vi "ELLjog.vi"() -> ()   [LabVIEW 2019]
uses:
  C:/Users/gboedecker/Downloads/ELL_Example/ELL/Thorlabs.Elliptec.ELLO_DLL.dll
  ELL_Example/ELL/Thorlabs.Elliptec.ELLO_DLL.dll
panel:
  out "Position":dbl format="%#.3f"
  in  "Enum":enum16{"None", "Button1", "Button2"}(ring)
  in  "Clockwise":bool
  in  "?":bool
  in  "Counter Clockwise":bool
  out "Connected":bool
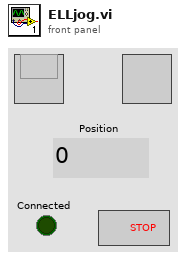
[diagram p1: front panel]
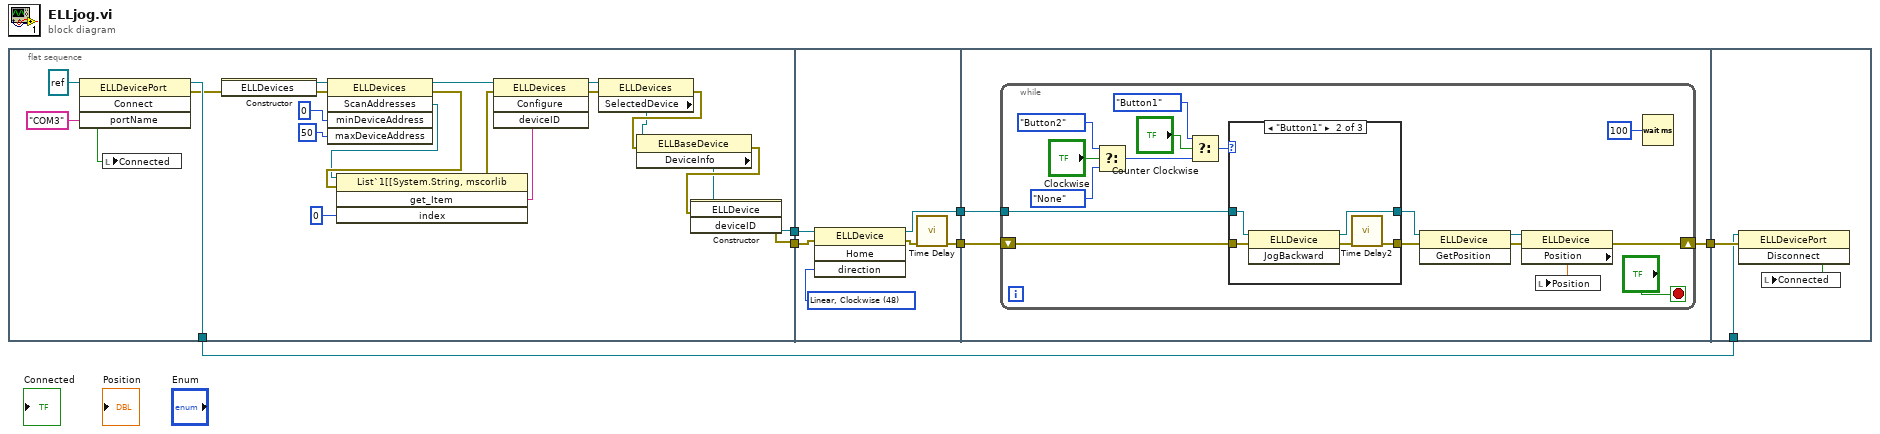
[diagram p0: block diagram]
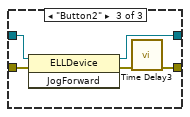
[diagram p3: hidden frame]
diagram:
  n1 = flat-sequence {
    tunnel: [w29] -> w3
    tunnel: [w28] -> w2
    tunnel: [w8] -> w1
    tunnel: [w35] -> w5
    tunnel: [w30] -> w4
    tunnel: w3 -> [w33]
    tunnel: w2 -> [w32]
    tunnel: [w38] -> w6
    tunnel: w5 -> [w37]
    tunnel: w4 -> [w36]
    tunnel: w6 -> [w69]
    tunnel: w1 -> [w68]
    frame #0 {
      n2 = invoke class="ELLDevicePort" method="Connect"(reference=refnum<k24> refnum, "portName"="COM3") -> (reference out=w8:refnum<k24>, error out=w7:errorcluster, "Connect"=w11:bool)  [unwired: 2 in, 1 out]
      n3 = local write "Connected"(w11) -> ()
      n4 = constructor class="ELLDevices"(error in=w7) -> (reference out=w13:refnum<k24>, error out=w12:errorcluster)  [unwired: 2 in, 1 out]
      n5 = invoke class="ELLDevices" method="ScanAddresses"(reference=w13, error in=w12, "minDeviceAddress"=u16 0, "maxDeviceAddress"=u16 50) -> (reference out=w16:refnum<k24>, error out=w15:errorcluster, "ScanAddresses"=w14:refnum<k24>)  [unwired: 1 in, 2 out]
      n6 = invoke class="List`1[[System.String, mscorlib" method="get_Item"(reference=w14, error in=w15, "index"=0) -> (error out=w21:errorcluster, "get_Item"=w20:string)  [unwired: 1 in, 2 out]
      n7 = invoke class="ELLDevices" method="Configure"(reference=w16, error in=w21, "deviceID"=w20) -> (reference out=w23:refnum<k24>, error out=w22:errorcluster)  [unwired: 1 in, 2 out]
      n8 = property class="ELLDevices"(reference=w23, error in=w22) -> (error out=w25:errorcluster, "SelectedDevice"=w24:refnum<k24>)  [unwired: 1 out]
      n9 = property class="ELLBaseDevice"(reference=w24, error in=w25) -> (error out=w27:errorcluster, "DeviceInfo"=w26:refnum<k24>)  [unwired: 1 out]
      n10 = constructor class="ELLDevice"(error in=w27, "deviceID"=w26) -> (reference out=w29:refnum<k24>, error out=w28:errorcluster)  [unwired: 2 in, 2 out]
    }
    frame #1 {
      w31 = 48 items=["Linear, Clockwise"=48, "AntiClockwise"=49] ("direction")
      n11 = invoke class="ELLDevice" method="Home"(reference=w33, error in=w32, "direction"=w31) -> (reference out=w35:refnum<k24>, error out=w34:errorcluster)  [unwired: 1 in, 2 out]
      n12 = call "Time Delay"("error in (no error)"=w34) -> ("error out"=w30:errorcluster)  [unwired: 10 in]
    }
    frame #2 {
      n13 = while {
        tunnel: w37 -> [w50]
        shift-right: [w53] -> w38
        shift-left: w36 -> [w49]
        stop <- "?" stop-if-true
        n14 = Select(t=enum16{"None", "Button1", "Button2"}."Button2" ("Enum"), s="Clockwise", f=enum16{"None", "Button1", "Button2"}."None" ("Enum")) -> (s? t:f=w43:enum16{"None", "Button1", "Button2"})
        n15 = Select(t=enum16{"None", "Button1", "Button2"}."Button1" ("Enum"), s="Counter Clockwise", f=w43) -> (s? t:f=w41:enum16{"None", "Button1", "Button2"})
        n16 = case shown="\"Button1\"" w41 {
          tunnel: [w56 w61 w63] -> w52
          tunnel: [w57 w60 w64] -> w51
          tunnel: w50 -> [w57 w59 w65]
          tunnel: w49 -> [w56 w58 w66]
          frame "None", Default {
          }
          frame "Button1" {
            n17 = invoke class="ELLDevice" method="JogBackward"(reference=w59, error in=w58) -> (reference out=w60:refnum<k24>, error out=w62:errorcluster)  [unwired: 1 in, 1 out]
            n18 = call "Time Delay2"("error in (no error)"=w62) -> ("error out"=w61:errorcluster)  [unwired: 10 in]
          }
          frame "Button2" {
            n19 = invoke class="ELLDevice" method="JogForward"(reference=w65, error in=w66) -> (reference out=w64:refnum<k24>, error out=w67:errorcluster)  [unwired: 1 in, 1 out]
            n20 = call "Time Delay3"("error in (no error)"=w67) -> ("error out"=w63:errorcluster)  [unwired: 10 in]
          }
        }
        n21 = invoke class="ELLDevice" method="GetPosition"(reference=w51, error in=w52) -> (reference out=w54:refnum<k24>, error out=w55:errorcluster)  [unwired: 1 in, 1 out]
        n22 = property class="ELLDevice"(reference=w54, error in=w55) -> (error out=w53:errorcluster, "Position"=w39:dbl)  [unwired: 1 out]
        n23 = local write "Position"(w39) -> ()
        n24 = Wait (ms)(milliseconds to wait=u32 100) -> ()  [unwired: 1 out]
      }
    }
    frame #3 {
      n25 = invoke class="ELLDevicePort" method="Disconnect"(reference=w68, error in=w69) -> ("Disconnect"=w70:bool)  [unwired: 1 in, 2 out]
      n26 = local write "Connected"(w70) -> ()
    }
  }
